vi "INL_Result.vi"(11 "Error In":errorcluster) -> (3 "Min INL Code":i32, 4 "Max INL Code":i32, 6 "Max INL":dbl format="%#.2e", 8 "INL Plot":cluster{"X":i32, "Y":dbl}[](graph), 10 "Min INL":dbl format="%#.2e", 15 "Error Out":errorcluster)   [LabVIEW 2026, in "Core.lvlib"]
doc: "Displays and summarizes the results of an INL measurement test, including graphical visualization and worst-case INL statistics."
uses:
  Core.lvlib
  TypeDefs/Enum_Events.ctl
  TypeDefs/Enum_Event_Options.ctl
  TypeDefs/Enum_Notifier_Name.ctl
  TypeDefs/Enum_Notifier_Options.ctl
panel:
  out "Total":i32
  out "Value":i32 caption="Currently processing value index:"
  # "/"
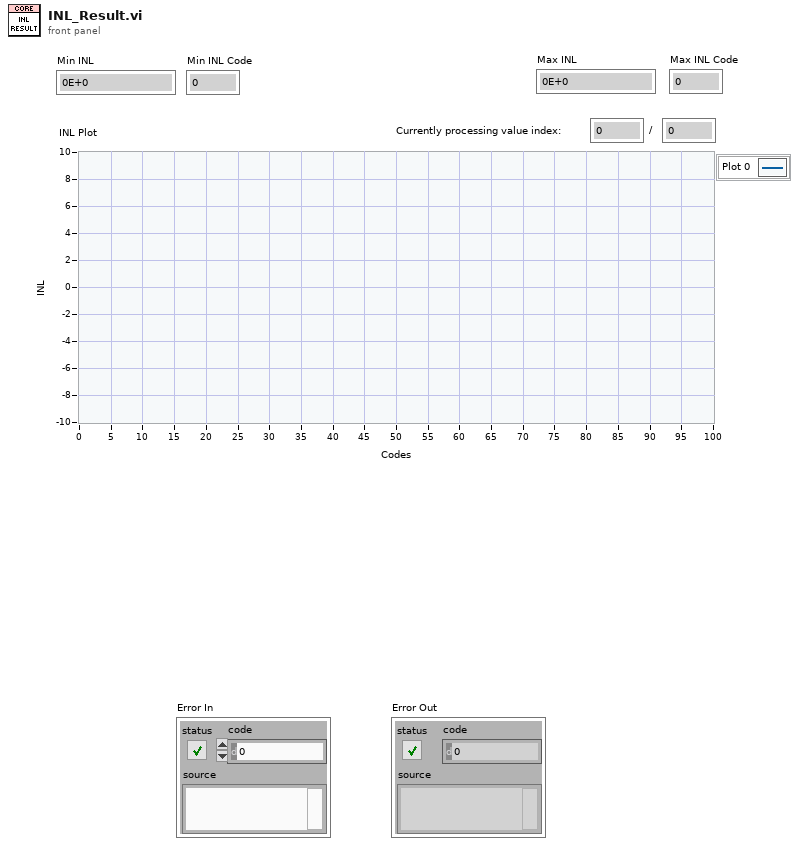
[diagram p1: front panel]
types:
  T1 = typedef "Core.lvlib/Enum_Notifier_Options.ctl" = enum16{"Create", "Send", "Status", "Release"}
  T2 = typedef "Core.lvlib/Enum_Notifier_Name.ctl" = enum16{"Device Type", "Test", "Instrument Spec", "Measurement Spec", "Status"}
  T3 = typedef "Core.lvlib/Enum_Event_Options.ctl" = enum16{"Create", "Generate", "Event Ref", "Destroy"}
  T4 = typedef "Core.lvlib/Enum_Events.ctl" = enum16{"Stop All", "Stop Subpanel", "Stop Test Spec", "Stop Result"}
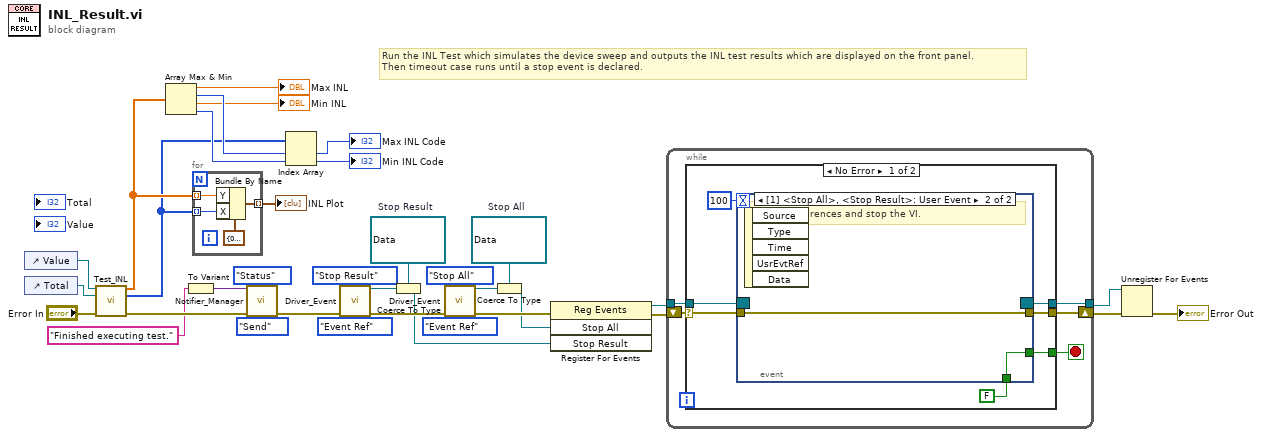
[diagram p0: block diagram]
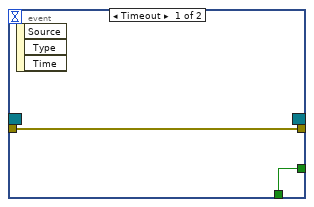
[diagram p2: hidden frame]
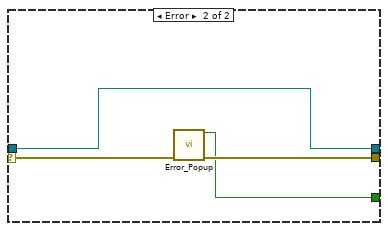
[diagram p3: hidden frame]
diagram:
  w16 = refnum<user-event> refnum  # Stop Result
  w18 = refnum<user-event> refnum  # Stop All
  # "Run the INL Test which simulates the device sweep and outputs the INL test results which are displayed on the front panel.\nThen timeout case runs until a stop event is declared."
  n1 = control-ref of="Value"() -> (w2:refnum<vi>)
  n2 = control-ref of="Total"() -> (w1:refnum<vi>)
  n3 = call "Test_INL.vi"("Value"=w2, "Total"=w1, "Error In"="Error In") -> ("INL"=w5:dbl[], "Codes Array"=w4:i32[], "Error Out"=w28:errorcluster)  [unwired: 10 in]
  n4 = Array Max & Min(array=w5) -> (max value=→"Max INL":dbl, max index (indices)=w33:i32, min value=→"Min INL":dbl, min index (indices)=w31:i32)
  n5 = To Variant(anything="Finished executing test.") -> (Variant=w6:variant)
  n6 = for {
    tunnel: w5 -> [w38] mode=indexing
    tunnel: w4 -> [w37] mode=indexing
    tunnel: [w36] -> w3 mode=indexing
    n7 = Bundle By Name(cluster=cluster{"X":i32, "Y":dbl} {"X"=0, "Y"=0.0}, "Y"=w38, "X"=w37) -> (w36:cluster{"X":i32, "Y":dbl})
  }
  "INL Plot" <- w3
  n8 = call "Notifier_Manager.vi"("Notifier Data"=w6, "Notifier Name"=Enum_Notifier_Name."Status", "Error In"=w28, "Notifier Options"=Enum_Notifier_Options."Send") -> ("Error Out"=w10:errorcluster)  [unwired: 10 in, 1 out]
  n9 = Index Array(array=w4, index #1=w33, index #2=w31) -> (element #1=→"Max INL Code":i32, element #2=→"Min INL Code":i32)
  n10 = call "Driver_Event.vi"("Event"=Enum_Events."Stop Result", "Error In"=w10, "Event Operation"=Enum_Event_Options."Event Ref") -> ("Event Ref"=w20:refnum<user-event>, "Error Out"=w23:errorcluster)  [unwired: 11 in]
  n11 = Coerce To Type(0:w20, 1:w16) -> (2:w17:refnum<user-event>)
  n12 = call "Driver_Event.vi"("Event"=Enum_Events."Stop All", "Error In"=w23, "Event Operation"=Enum_Event_Options."Event Ref") -> ("Event Ref"=w21:refnum<user-event>, "Error Out"=w22:errorcluster)  [unwired: 11 in]
  n13 = Coerce To Type(0:w21, 1:w18) -> (2:w19:refnum<user-event>)
  n14 = register-events(error in=w22, w19, w17) -> (reference out=w14:refnum<event-registration>, error out=w15:errorcluster)  [unwired: 1 in]
  n15 = while {
    tunnel: w14 -> [w41]
    shift-right: [w43] -> w13
    shift-left: w15 -> [w44]
    tunnel: [w40] -> w11
    stop <- w42 stop-if-true
    n16 = case shown="No Error" w44 {
      selector: w44 -> [w50 w59]
      tunnel: [w49 w58] -> w43
      tunnel: [w48 w57] -> w42
      tunnel: w41 -> [w46 w56]
      tunnel: [w45 w56] -> w40
      frame No Error {
        n17 = event shown="[1] <Stop All>, <Stop Result>: User Event" {
          selector: w46 -> [_ _]
          dyn-events: [_ _] -> w45
          timeout: 100 -> [_ _]
          tunnel: w50 -> [w53 w55]
          tunnel: [w53 w55] -> w49
          tunnel: [w52 w54] -> w48
          tunnel: FALSE -> [w52 w54]
          event Timeout {
            n18 = event-data() -> ()  [unwired: 1 in, 3 out]
          }
          event User Event {
            # "Close all references and stop the VI."
            n19 = event-data() -> ()  [unwired: 1 in, 5 out]
          }
        }
      }
      frame Error {
        n20 = call "Error_Popup.vi"("Error In"=w59) -> ("Stop?"=w57:bool, "Error Out"=w58:errorcluster)  [unwired: 13 in]
      }
    }
  }
  n21 = Unregister For Events(event registration refnum=w11, error in=w13) -> (error out=→"Error Out":errorcluster)
